vi "RemoteVI Complex Fixture Refs.vi"(0 "Controls":refnum<vi>[](array[refnum])) -> (4 "Settings Ref":refnum<vi>, 5 "Rate Ref":refnum<vi>, 6 "Level Ref":refnum<vi>, 7 "Nav Ref":refnum<vi>, 8 "Scope Ref":refnum<vi>, 9 "Channel Ref":refnum<vi>, 10 "Results Ref":refnum<vi>, 11 "Steps Ref":refnum<vi>)   [LabVIEW 2020]
doc: "Helper of RemoteVI Complex Fixture Events.vi. Splits the array of control references RemoteVI Complex Fixture Find Controls.vi returns for Settings, Rate, Level, Nav, Scope, Channel, Results, Steps into one named reference each, so Register For Events names each event source after its control (<Settings Ref>)."
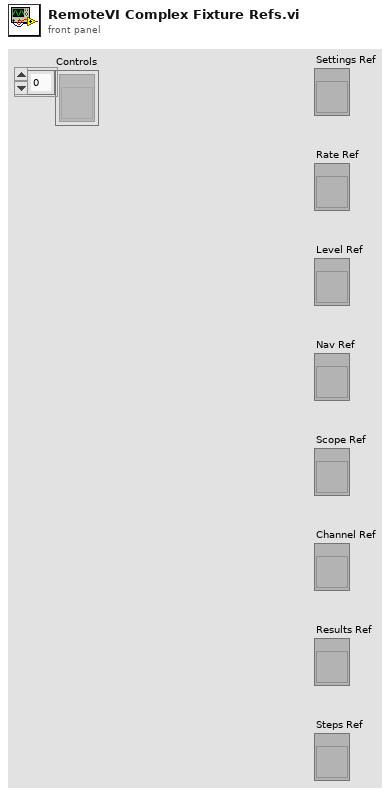
[diagram p1: front panel]
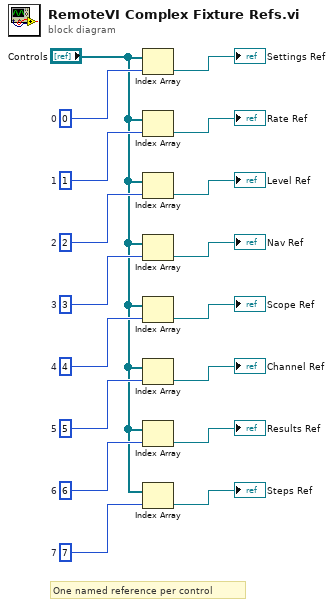
[diagram p0: block diagram]
diagram:
  w16 = 7  # 7
  w14 = 6  # 6
  w12 = 5  # 5
  w10 = 4  # 4
  w8 = 3  # 3
  w6 = 2  # 2
  w4 = 1  # 1
  w2 = 0  # 0
  # "One named reference per control"
  n1 = Index Array(array="Controls", index=w2) -> (element=→"Settings Ref":refnum<vi>)
  n2 = Index Array(array="Controls", index=w4) -> (element=→"Rate Ref":refnum<vi>)
  n3 = Index Array(array="Controls", index=w6) -> (element=→"Level Ref":refnum<vi>)
  n4 = Index Array(array="Controls", index=w8) -> (element=→"Nav Ref":refnum<vi>)
  n5 = Index Array(array="Controls", index=w10) -> (element=→"Scope Ref":refnum<vi>)
  n6 = Index Array(array="Controls", index=w12) -> (element=→"Channel Ref":refnum<vi>)
  n7 = Index Array(array="Controls", index=w14) -> (element=→"Results Ref":refnum<vi>)
  n8 = Index Array(array="Controls", index=w16) -> (element=→"Steps Ref":refnum<vi>)
